vi "Reset Fault.vi"(8 "error in (no error)":errorcluster, 11 "WEG_SCA06_Modbus in":refnum<class "WEG_SCA06_Modbus.lvclass">) -> (0 "error out":errorcluster, 3 "WEG_SCA06_Modbus out":refnum<class "WEG_SCA06_Modbus.lvclass">)   [LabVIEW 2021, in "WEG_SCA06_Modbus.lvclass"]
uses:
  WEG_SCA06_Modbus.lvclass
  WEG_SCA06_Modbus.lvclass/WEG_SCA06_Modbus.ctl
  Modbus_Master/Modbus_Master.lvclass
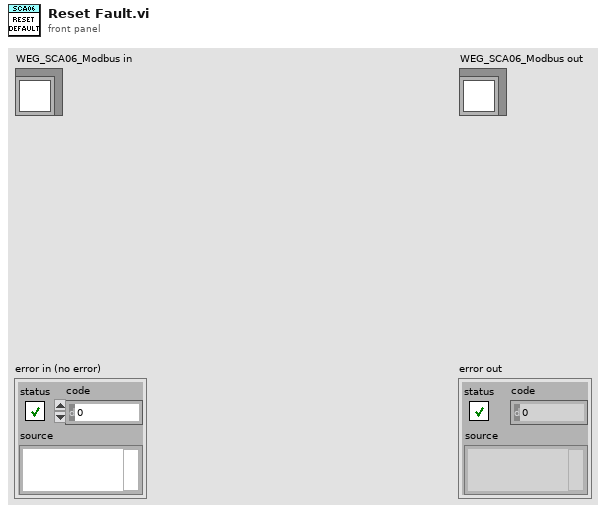
[diagram p1: front panel]
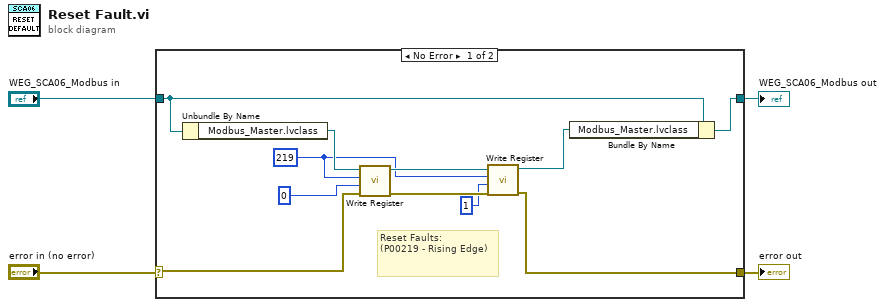
[diagram p0: block diagram]
diagram:
  n1 = case shown="No Error" "error in (no error)" {
    selector: "error in (no error)" -> [w12 w17]
    tunnel: [w8 w17] -> w3
    tunnel: [w15 w16] -> w2
    tunnel: "WEG_SCA06_Modbus in" -> [w14 w16]
    frame No Error {
      w6 = u16 219 ("Register Address")
      # "Reset Faults:\n(P00219 - Rising Edge)"
      n2 = Unbundle By Name(w14) -> ("Modbus_Master.lvclass"=w13:refnum<class "Modbus_Master.lvclass">)
      n3 = call "Write Register.vi"("error in (no error)"=w12, "Value"=u16 0, "Register Address"=w6, "Modbus_Master in"=w13) -> ("error out"=w10:errorcluster, "Modbus_Master out"=w11:refnum<class "Modbus_Master.lvclass">)  [unwired: 6 in]
      n4 = call "Write Register.vi"("error in (no error)"=w10, "Value"=u16 1, "Register Address"=w6, "Modbus_Master in"=w11) -> ("error out"=w8:errorcluster, "Modbus_Master out"=w9:refnum<class "Modbus_Master.lvclass">)  [unwired: 6 in]
      n5 = Bundle By Name(cluster=w14, "Modbus_Master.lvclass"=w9) -> (w15:refnum<class "WEG_SCA06_Modbus.lvclass">)
    }
    frame Error {
    }
  }
  "error out" <- w3
  "WEG_SCA06_Modbus out" <- w2
